vi "CSE ISP - validate callback VI path.vi"(9 "Old Path":path, 10 "New Path":path, 11 "Path Refnum":refnum<vi>) -> ()   [LabVIEW 2021]
doc: "::: CalcExpress Toolkit :::\nCopyright (c) 2000-2026 Konstantin Shifershteyn. All rights reserved."
uses:
  vi.lib/addons/CalcExpress/cse.llb/CSE Callback VI RefNum.ctl
panel:
  in  "Callback VI RefNum":T1
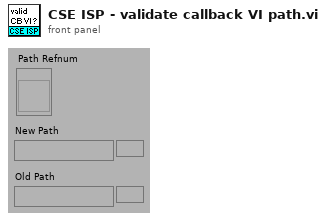
[diagram p1: front panel]
types:
  T1 = typedef "CSE Callback VI RefNum.ctl" = refnum<vi>
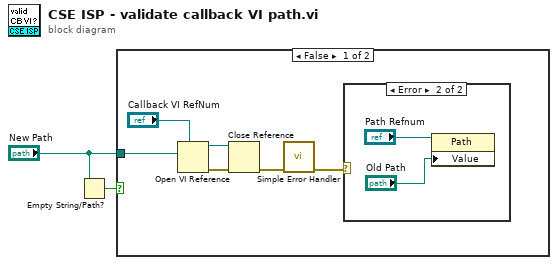
[diagram p0: block diagram]
diagram:
  n1 = Empty String/Path?(string/path="New Path") -> (empty?=w2:bool)
  n2 = case shown="False" w2 {
    tunnel: "New Path" -> [w5 _]
    frame False {
      n3 = Open VI Reference(type specifier VI Refnum (for type only)="Callback VI RefNum", vi path=w5) -> (vi reference=w8:T1, error out=w7:errorcluster)  [unwired: 4 in]
      n4 = Close Reference(reference=w8, error in (no error)=w7) -> (error out=w6:errorcluster)
      n5 = call <vilib>:"Simple Error Handler.vi"("error in (no error)"=w6) -> ("error out"=w3:errorcluster)  [unwired: 4 in, 4 out]
      n6 = case shown="Error" w3 {
        frame No Error {
        }
        frame Error {
          n7 = property class="Path"(reference="Path Refnum", "Value"="Old Path") -> ()  [unwired: 1 in, 2 out]
        }
      }
    }
    frame True {
    }
  }
